vi "Sous_VI_correction.vi"(8 "error in (no error)":errorcluster, 10 "G/D ?":bool, 11 "Décalage":u32(graph)) -> (0 "error out":errorcluster)   [LabVIEW 2018]
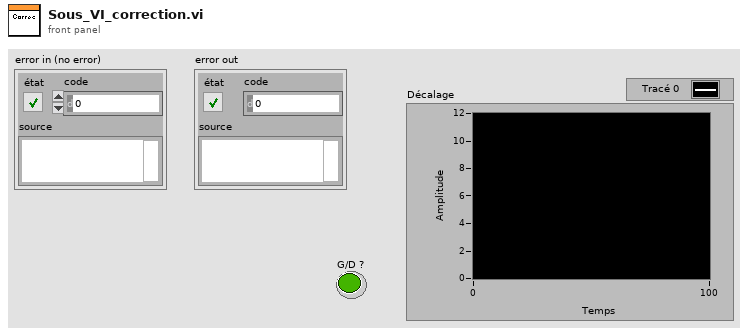
[diagram p1: front panel]
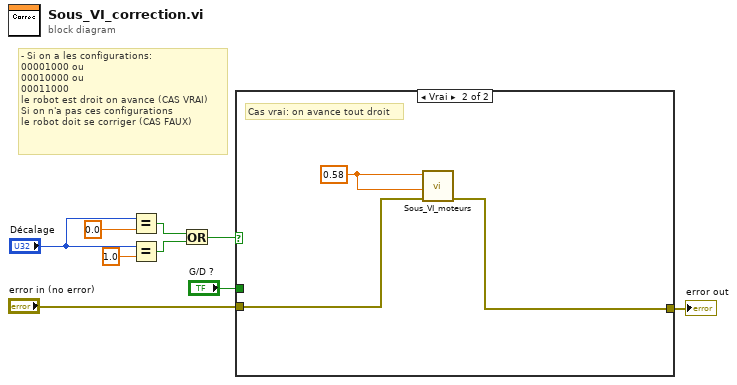
[diagram p0: block diagram]
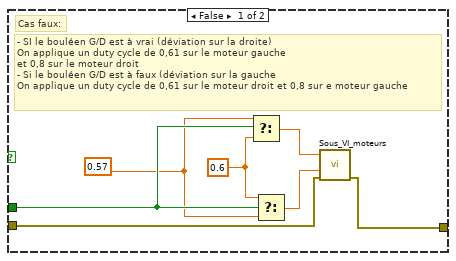
[diagram p2: hidden frame]
diagram:
  # "- Si on a les configurations:\n00001000 ou\n00010000 ou\n00011000\nle robot est droit on avance (CAS VRAI)\nSi on n'a pas ces configurations\nle robot doit se corriger (CAS FAUX)"
  n1 = Equal?(x="Décalage", y=0.0) -> (x = y?=w7:bool)
  n2 = Equal?(x="Décalage", y=1.0) -> (x = y?=w6:bool)
  n3 = Or(x=w7, y=w6) -> (x .or. y?=w5:bool)
  n4 = case shown="Vrai" w5 {
    tunnel: "G/D ?" -> [w14 _]
    tunnel: "error in (no error)" -> [w11 w19]
    tunnel: [w10 w17] -> w1
    frame False {
      w13 = 0.57 ("cas vrai")
      w16 = 0.6 ("cas faux")
      # "Cas faux:"
      # "- SI le bouléen G/D est à vrai (déviation sur la droite)\nOn applique un duty cycle de 0,61 sur le moteur gauche\net 0,8 sur le moteur droit\n- Si le bouléen G/D est à faux (déviation sur la gauche\nOn applique un duty cycle de 0,61 sur le moteur droit et 0,8 sur e moteur gauche"
      n5 = Select(t=w13, s=w14, f=w16) -> (s? t:f=w15:dbl)
      n6 = Select(t=w16, s=w14, f=w13) -> (s? t:f=w12:dbl)
      n7 = call "Sous_VI_moteurs.vi"("error in (no error)"=w11, "Moteur Droit"=w12, "Moteur Gauche"=w15) -> ("error out"=w10:errorcluster)  [unwired: 8 in]
    }
    frame True {
      w18 = 0.58
      # "Cas vrai: on avance tout droit"
      n8 = call "Sous_VI_moteurs.vi"("error in (no error)"=w19, "Moteur Droit"=w18, "Moteur Gauche"=w18) -> ("error out"=w17:errorcluster)  [unwired: 8 in]
    }
  }
  "error out" <- w1
